vi "flush batch buffer.vi"(10 "batch buffer":refnum<data-value>, 11 "stream session":refnum<data-value>) -> (0 "error out":errorcluster)   [LabVIEW 2020, in "nominal core steps.lvlib"]
doc: "Flushes all stored data to a stream."
uses:
  nominal core steps.lvlib
  batch buffer.ctl
  channel uid.ctl
  points buffer.ctl
  single point.ctl
  stream session.ctl
  <vilib>/Nominal/Nominal IO Client/submodules/nominal-streaming-labview-ffi/lv_src/Stream/Stream.lvclass
  <vilib>/Nominal/Nominal IO Client/submodules/nominal-streaming-labview-ffi/lv_src/Channel/Channel.lvclass
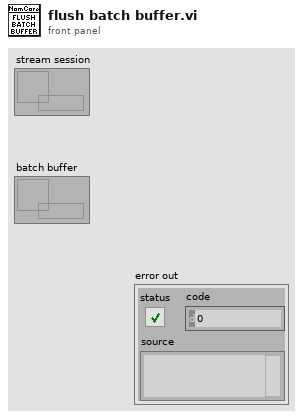
[diagram p1: front panel]
types:
  T1 = typedef "nominal core steps.lvlib/batch buffer.ctl" = map{T2, refnum<data-value>}
  T2 = typedef "nominal core steps.lvlib/channel uid.ctl" = cluster{"channel name":string, "tags":map{string, string}}
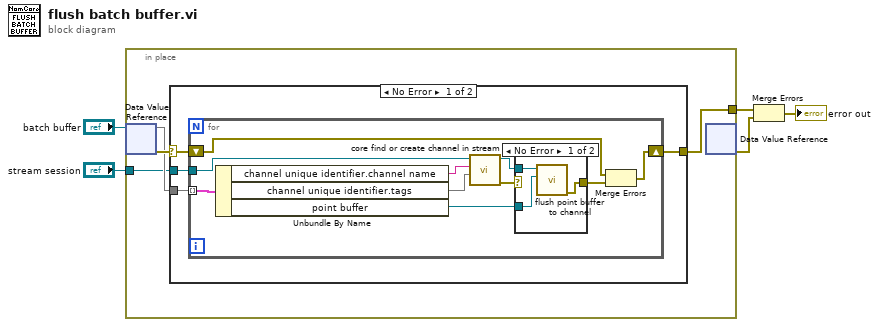
[diagram p0: block diagram]
diagram:
  n1 = in-place {
    in-place-border: [w8] -> w4
    in-place-border: "stream session" -> [w6]
    n2 = in-place-dvr #1("batch buffer") -> (w7:T1, w9:errorcluster)
    n3 = case shown="No Error" w9 {
      selector: w9 -> [w12 w28]
      tunnel: [w11 w28] -> w8
      tunnel: w7 -> [w10 _]
      tunnel: w6 -> [w13 _]
      frame No Error {
        n4 = for {
          tunnel: w10 -> [w23] mode=indexing
          tunnel: w13 -> [w18]
          shift-right: [w21] -> w11
          shift-left: w12 -> [w22]
          n5 = Unbundle By Name(w23) -> ("channel unique identifier.channel name"=w17:string, "channel unique identifier.tags"=w16:map{string, string}, "point buffer"=w20:refnum<data-value>)
          n6 = call "core find or create channel in stream.vi"("tags"=w16, "channel name"=w17, "stream"=w18) -> ("error out"=w14:errorcluster, "channel"=w15:refnum<class "Channel.lvclass">)  [unwired: 7 in]
          n7 = case shown="No Error" w14 {
            selector: w14 -> [_ w27]
            tunnel: w20 -> [w26 _]
            tunnel: [w25 w27] -> w19
            tunnel: w15 -> [w24 _]
            frame No Error {
              n8 = call "flush point buffer to channel.vi"("point buffer"=w26, "channel"=w24) -> ("error out"=w25:errorcluster)  [unwired: 9 in]
            }
            frame Error {
            }
          }
          n9 = Merge Errors(w22, w19) -> (w21:errorcluster)
        }
      }
      frame Error {
      }
    }
    n10 = in-place-dvr #1() -> (w3:errorcluster)  [unwired: 1 in, 1 out]
  }
  n11 = Merge Errors(w4, w3) -> (→"error out":errorcluster)
